vi "labview-quick-video.vi"   [LabVIEW 2020]
uses:
  Nominal Client/Nominal Client.lvclass/Nominal Client.ctl
  User/User.lvclass
  Nominal Client/Nominal Client.lvclass
  nominal types/workspace/workspace.lvclass
  submodules/reqwest-labview/lv-src/reqwest/reqwest.lvclass
  e79185ee-863a-4b48-b269-365b27d9e424.vi
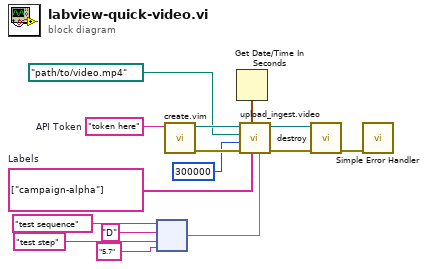
[diagram p0: block diagram]
diagram:
  w4 = string[] ["campaign-alpha"]  # Labels
  w14 = "token here"  # API Token
  n1 = node("test sequence", "D", "test step", "5.7") -> (w3:map{string, string})
  n2 = call "create.vim"("API Token (string or path)"=w14) -> ("error out"=w7:errorcluster, "Nominal Client"=w9:refnum<class "Nominal Client.lvclass">)  [unwired: 8 in, 1 out]
  n3 = Get Date/Time In Seconds() -> (seconds since 1Jan1904=w2:timestamp)
  n4 = call "upload_ingest.video.vi"("Properties"=w3, "Labels"=w4, "Time Stamp"=w2, "error in"=w7, "timeout (ms)"=300000, "File Path"=path "path/to/video.mp4", "Nominal Client in"=w9) -> ("error out"=w6:errorcluster, "Nominal Client out"=w8:refnum<class "Nominal Client.lvclass">)  [unwired: 2 in, 1 out]
  n5 = call "destroy.vi"("error in"=w6, "Nominal Client"=w8) -> ("error out"=w15:errorcluster)  [unwired: 9 in]
  n6 = call <vilib>:"Simple Error Handler.vi"("error in (no error)"=w15) -> ()  [unwired: 4 in, 5 out]
